vi "Register.vi"(8 "error in (no error)":errorcluster, 11 "logger in":refnum<class "Logger.lvclass">) -> (0 "error out":errorcluster)   [LabVIEW 2018, in "GLog.lvlib" / "Registry.lvlib"]
uses:
  Registry.lvlib
  api/logger_class/Logger.lvclass
  Registry Actions.ctl
  Register Action Data.ctl
panel:
  # "Connector Pane"
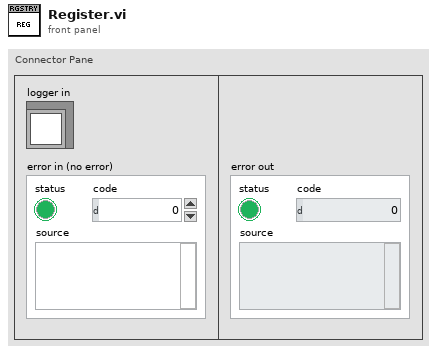
[diagram p1: front panel]
types:
  T1 = typedef "GLog.lvlib/Registry.lvlib/Register Action Data.ctl" = cluster{"Logger":refnum<class "Logger.lvclass">, "Owning VI":string}
  T2 = typedef "GLog.lvlib/Registry.lvlib/Registry Actions.ctl" = enum16{"Register", "Log", "Enable", "Enable All", "Disable", "Disable All", "Get Enable State", "Get Minimum Log Level", "Set Minimum Log Level", "Set All Minimum Log Level", "Get Logger Info", "Get All Logger Info", "List", "Unregister", "Unregister All", "Shutdown"}
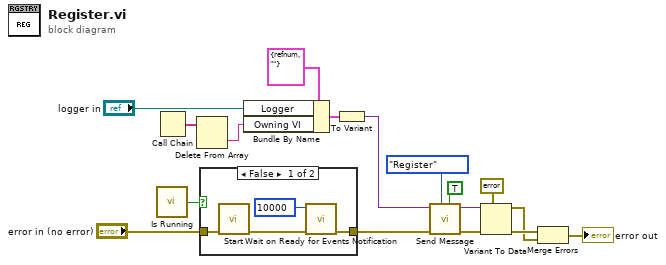
[diagram p0: block diagram]
diagram:
  n1 = call "Is Running.vi"() -> ("is running?"=w1:bool)  [unwired: 1 in]
  n2 = Call Chain() -> (call chain=w6:string[])
  n3 = Delete From Array(array=w6) -> (deleted portion=w5:string)  [unwired: 2 in, 1 out]
  n4 = case shown="False" w1 {
    tunnel: "error in (no error)" -> [w19 w22]
    tunnel: [w18 w22] -> w12
    frame False {
      n5 = call "Start.vi"("error in (no error)"=w19) -> ("error out"=w20:errorcluster)  [unwired: 10 in]
      n6 = call "Wait on Ready for Events Notification.vi"("error in (no error)"=w20, "timeout [ms]"=10000 ("timeout in ms (-1)")) -> ("error out"=w18:errorcluster)  [unwired: 9 in]
    }
    frame True {
    }
  }
  n7 = Bundle By Name(cluster=T1 {"Logger"=refnum, "Owning VI"=""} ("Logging.lvlib:Logger.lvclass"), "Logger"="logger in", "Owning VI"=w5) -> (w4:T1)
  n8 = To Variant(anything=w4) -> (Variant=w16:variant)
  n9 = call "Send Message.vi"("return data? (F)"=TRUE, "action"=Registry_Actions."Register", "error in (no error)"=w12, "send data"=w16) -> ("error out"=w11:errorcluster, "Variant"=w14:variant)  [unwired: 6 in]
  n10 = Variant To Data(error in=w11, type=errorcluster {"status"=FALSE, "code"=0, "source"=""} ("error in (no error)"), Variant=w14) -> (data=w9:errorcluster, error out=w10:errorcluster)
  n11 = Merge Errors(w10, w9) -> (→"error out":errorcluster)
